vi "wait on clock.vi"(8 "error in":errorcluster, 10 "dt":u32=1, 11 "timing source in":refnum<class "usec timing source.lvclass">) -> (0 "error out":errorcluster, 2 "ticks since last call":u32, 3 "timing source out":refnum<class "usec timing source.lvclass">)   [LabVIEW 2013, in "usec timing source.lvclass"]
doc: "This core timing function is used inside of a loop to wait for a clock signal, or dt ticks of a clock signal."
uses:
  usec timing source.lvclass
  usec timing source.lvclass/usec timing source.ctl
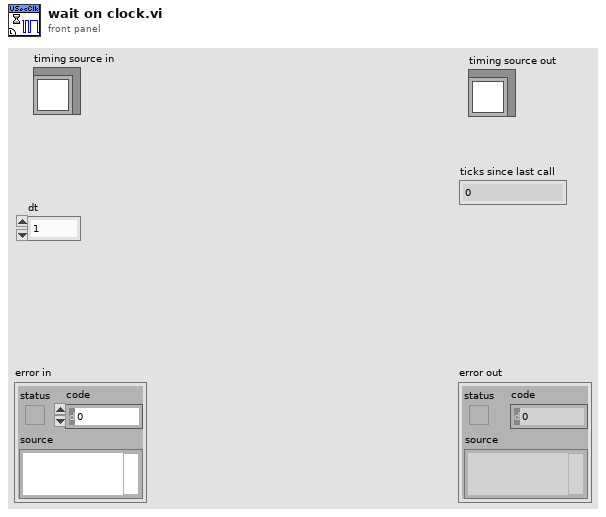
[diagram p1: front panel]
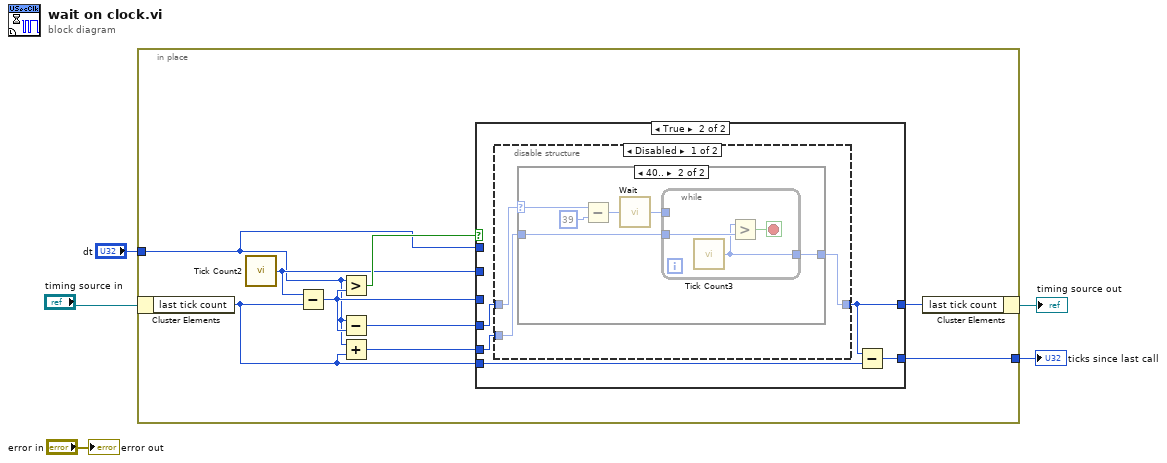
[diagram p0: block diagram]
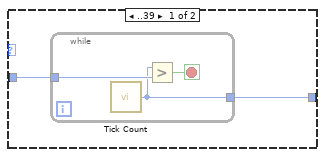
[diagram p3: hidden frame]
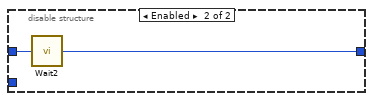
[diagram p4: hidden frame]
diagram:
  n1 = in-place {
    in-place-border: [w11] -> w4
    in-place-border: "dt" -> [w7]
    n2 = in-place-cluster #1("timing source in") -> ("last tick count"=w6:u32)
    n3 = call "Tick Count2"() -> ("Tick Count(uSec)"=w12:u32)
    n4 = Subtract(x=w12, y=w6) -> (x-y=w10:u32)
    n5 = Greater?(x=w7, y=w10) -> (0:w14:bool)
    n6 = Subtract(x=w7, y=w10) -> (x-y=w9:u32)
    n7 = Add(x=w7, y=w6) -> (x+y=w8:u32)
    n8 = case shown="True" w14 {
      tunnel: [w16 w19] -> w13
      tunnel: w12 -> [w16 _]
      tunnel: [w15 w18] -> w11
      tunnel: w10 -> [w15 _]
      tunnel: w9 -> [_ w21]
      tunnel: w8 -> [_ w20]
      tunnel: w7 -> [_ _]
      tunnel: w6 -> [_ w17]
      frame False {
      }
      frame True {
        n9 = disable-structure shown="Disabled" {
          disable-tunnel: w21 -> [w24 w40]
          disable-tunnel: w20 -> [w23 _]
          disable-tunnel: [w22 w39] -> w19
          frame Disabled {
            n10 = case shown="40.." w24 {
              selector: w24 -> [_ w35]
              tunnel: w23 -> [w26 w32]
              tunnel: [w25 w31] -> w22
              frame ..39 {
                n11 = while {
                  tunnel: w26 -> [w29]
                  tunnel: [w27] -> w25
                  stop <- w28 stop-if-true
                  n12 = call "Tick Count"() -> ("Tick Count(uSec)"=w27:u32)
                  n13 = Greater?(x=w27, y=w29) -> (0:w28:bool)
                }
              }
              frame 40.. {
                n14 = Subtract(x=w35, y=u32 39) -> (x-y=w33:u32)
                n15 = call "Wait"("Count(uSec)"=w33) -> ("Tick Count(uSec)"=w30:u32)
                n16 = while {
                  tunnel: w32 -> [w38]
                  tunnel: [w36] -> w31
                  tunnel: w30 -> [_]
                  stop <- w37 stop-if-true
                  n17 = call "Tick Count3"() -> ("Tick Count(uSec)"=w36:u32)
                  n18 = Greater?(x=w36, y=w38) -> (0:w37:bool)
                }
              }
            }
          }
          frame Enabled {
            n19 = call "Wait2"("Count(uSec)"=w40) -> ("Tick Count(uSec)"=w39:u32)
          }
        }
        n20 = Subtract(x=w19, y=w17) -> (x-y=w18:u32)
      }
    }
    n21 = in-place-cluster #1("last tick count"=w13) -> (→"timing source out":refnum<class "usec timing source.lvclass">)
  }
  "ticks since last call" <- w4
  "error out" <- "error in"
